vi "test_GetItemInfosFromProjectFile_SampleProject.vi"() -> (3 "Pass?":bool)   [LabVIEW 2019, in "Tests.SolutionBuilder.lvlib"]
uses:
  Tests.SolutionBuilder.lvlib
  SolutionBuilder/SolutionBuilder.lvclass
  SolutionBuilder/ProjectItem/ProjectItem.lvclass
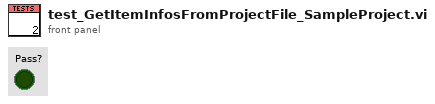
[diagram p1: front panel]
types:
  T1 = typedef "SolutionBuilder.lvlib/SolutionBuilder.lvclass/ProjectItemMap.ctl" = map{path, refnum<class "ProjectItem.lvclass">[]}
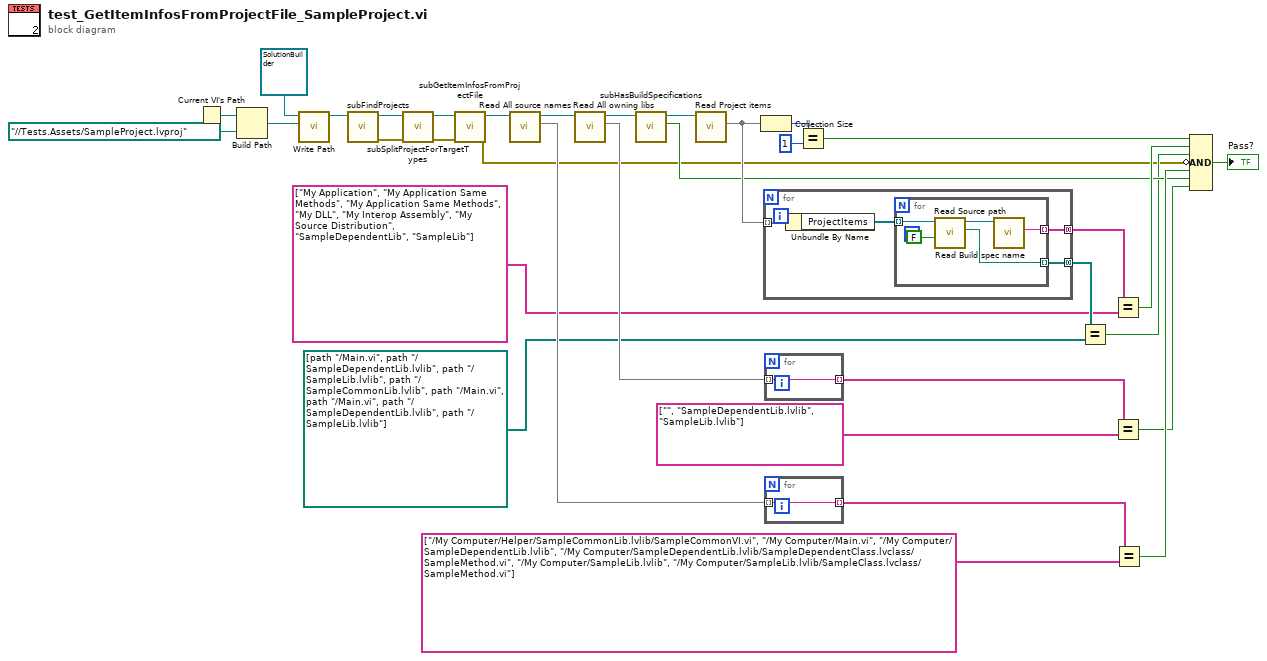
[diagram p0: block diagram]
diagram:
  n1 = Current VI's Path() -> (path=w32:path)
  n2 = Build Path(base path=w32, name or relative path=path "../../Tests.Assets/SampleProject.lvproj" ("Path")) -> (appended path=w30:path)
  n3 = call "Write Path.vi"("Path"=w30, "SolutionBuilder in"=refnum<class "SolutionBuilder.lvclass"> refnum) -> ("SolutionBuilder out"=w33:refnum<class "SolutionBuilder.lvclass">)  [unwired: 9 in]
  n4 = call "subFindProjects.vi"("SolutionBuilder in"=w33) -> ("error out"=w3:errorcluster, "SolutionBuilder out"=w4:refnum<class "SolutionBuilder.lvclass">)  [unwired: 9 in]
  n5 = call "subSplitProjectForTargetTypes.vi"("error in (no error)"=w3, "SolutionBuilder in"=w4) -> ("error out"=w2:errorcluster, "SolutionBuilder out"=w1:refnum<class "SolutionBuilder.lvclass">)  [unwired: 8 in]
  n6 = call "subGetItemInfosFromProjectFile.vi"("error in (no error)"=w2, "SolutionBuilder in"=w1) -> ("error out"=w6:errorcluster, "SolutionBuilder out"=w27:refnum<class "SolutionBuilder.lvclass">)  [unwired: 8 in]
  n7 = call "Read All source names.vi"("SolutionBuilder in"=w27) -> ("All source names"=w23:set{string}, "SolutionBuilder out"=w14:refnum<class "SolutionBuilder.lvclass">)  [unwired: 9 in]
  n8 = call "Read All owning libs.vi"("SolutionBuilder in"=w14) -> ("All owning libs"=w12:set{string}, "SolutionBuilder out"=w13:refnum<class "SolutionBuilder.lvclass">)  [unwired: 9 in]
  n9 = call "subHasBuildSpecifications.vi"("SolutionBuilder in"=w13) -> ("Has specs?"=w20:bool, "SolutionBuilder out"=w21:refnum<class "SolutionBuilder.lvclass">)  [unwired: 8 in, 1 out]
  n10 = call "Read Project items.vi"("SolutionBuilder in"=w21) -> ("Project items"=w26:T1)  [unwired: 9 in, 1 out]
  n11 = Collection Size(1:w26) -> (0:w29:i32)
  n12 = for {
    tunnel: w26 -> [w38] mode=indexing
    tunnel: [w37] -> w19 mode=concatenating
    tunnel: [w35] -> w16 mode=concatenating
    n13 = Unbundle By Name(w38) -> ("ProjectItems"=w36:refnum<class "ProjectItem.lvclass">[])
    n14 = for {
      tunnel: w36 -> [w41] mode=indexing
      tunnel: [w43] -> w37 mode=indexing
      tunnel: [w40] -> w35 mode=indexing
      n15 = call "Read Source path.vi"("Force abs path? (T)"=FALSE, "ProjectItem in"=w41) -> ("Source path"=w40:path, "ProjectItem out"=w42:refnum<class "ProjectItem.lvclass">)  [unwired: 8 in]
      n16 = call "Read Build spec name.vi"("ProjectItem in"=w42) -> ("Build spec name"=w43:string)  [unwired: 9 in, 1 out]
    }
  }
  n17 = for {
    tunnel: w12 -> [w44] mode=indexing
    tunnel: [w44] -> w11 mode=indexing
  }
  n18 = for {
    tunnel: w23 -> [w45] mode=indexing
    tunnel: [w45] -> w18 mode=indexing
  }
  n19 = Equal?(x=w29, y=1) -> (x = y?=w25:bool)
  n20 = Equal?(x=w16, y=path[] [path "../Main.vi", path "../SampleDependentLib.lvlib", path "../SampleLib.lvlib", path "../SampleCommonLib.lvlib", path "../Main.vi", path "../Main.vi", path "../SampleDependentLib.lvlib", path "../SampleLib.lvlib"] ("Array 2")) -> (x = y?=w15:bool)
  n21 = Equal?(x=w19, y=string[] ["My Application", "My Application Same Methods", "My Application Same Methods", "My DLL", "My Interop Assembly", "My Source Distribution", "SampleDependentLib", "SampleLib"] ("Array")) -> (x = y?=w24:bool)
  n22 = Equal?(x=w11, y=string[] ["", "SampleDependentLib.lvlib", "SampleLib.lvlib"] ("Array")) -> (x = y?=w9:bool)
  n23 = Equal?(x=w18, y=string[] ["/My Computer/Helper/SampleCommonLib.lvlib/SampleCommonVI.vi", "/My Computer/Main.vi", "/My Computer/SampleDependentLib.lvlib", "/My Computer/SampleDependentLib.lvlib/SampleDependentClass.lvclass/SampleMethod.vi", "/My Computer/SampleLib.lvlib", "/My Computer/SampleLib.lvlib/SampleClass.lvclass/SampleMethod.vi"] ("Array 2")) -> (x = y?=w22:bool)
  n24 = Compound Arithmetic op=AND(w25, w24, w15, invert w6, w22, w20, w9) -> (→"Pass?":bool)
